vi "lab2_3.vi"() -> ()   [LabVIEW 2026]
uses:
  <vilib>/eio/EIONode/EIONode.xnode
  <vilib>/rvi/eio/common/nirviEmuTemplateMethod_errors.vi
panel:
  out "Mean X":fxp<+/-,64,33>
  out "AccelerationZ Now":i16
  out "AccelerationZ Max":i16
  out "AccelerationY Max":i16
  out "AccelerationY Now":i16
  out "AccelerationX Max":i16
  out "AccelerationX Now":i16
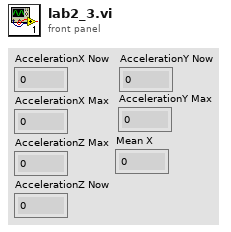
[diagram p1: front panel]
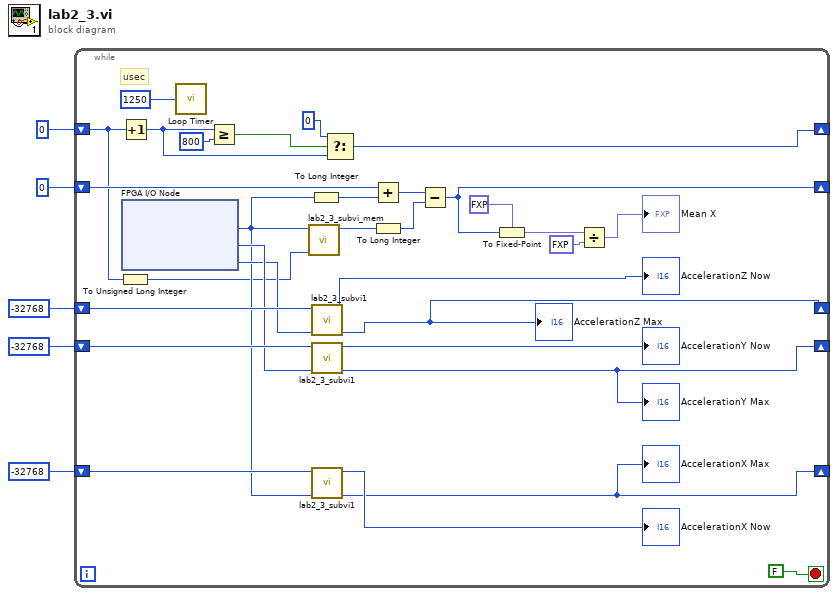
[diagram p0: block diagram]
diagram:
  n1 = while {
    shift-right: [w25] -> _
    shift-left: i16 -32768 ("x") -> [w30]
    shift-right: [w32] -> _
    shift-left: i16 -32768 ("x") -> [w34]
    shift-right: [w26] -> _
    shift-left: i16 -32768 ("x") -> [w31]
    shift-right: [w13] -> _
    shift-left: 0 ("x") -> [w23]
    shift-right: [w7] -> _
    shift-left: 0 ("x") -> [w6]
    stop <- FALSE stop-if-true
    # "usec"
    n2 = To Unsigned Long Integer(number=w6) -> (unsigned 32bit integer=w14:u32)
    n3 = Increment(x=w6) -> (x+1=w8:i32)
    n4 = xnode "FPGA I/O Node"() -> ("AccelerationX"=w21:i16, "AccelerationY"=w29:i16, "AccelerationZ"=w28:i16)  [unwired: 3 in, 3 out]
    n5 = call "Loop Timer"("Count(uSec)"=u32 1250) -> ()  [unwired: 1 out]
    n6 = Greater Or Equal?(x=w8, y=800) -> (x >= y?=w16:bool)
    n7 = call "lab2_3_subvi_mem.vi"("Address"=w14, "Data In"=w21) -> ("Last Value"=w19:i16)  [unwired: 9 in]
    n8 = To Long Integer(number=w21) -> (32bit integer=w22:i32)
    n9 = call "lab2_3_subvi1.vi"("Acc in"=w28, "Acc prev"=w30) -> ("Acceleration Max"=w25:i16, "Acceleration Now"=→"AccelerationZ Now":i16)  [unwired: 8 in]
    "AccelerationZ Max" <- w25
    n10 = call "lab2_3_subvi1.vi"("Acc in"=w29, "Acc prev"=w31) -> ("Acceleration Max"=w26:i16, "Acceleration Now"=→"AccelerationY Now":i16)  [unwired: 8 in]
    "AccelerationY Max" <- w26
    n11 = call "lab2_3_subvi1.vi"("Acc in"=w21, "Acc prev"=w34) -> ("Acceleration Max"=w32:i16, "Acceleration Now"=→"AccelerationX Now":i16)  [unwired: 8 in]
    "AccelerationX Max" <- w32
    n12 = Select(t=0, s=w16, f=w8) -> (s? t:f=w7:i32)
    n13 = Add(x=w23, y=w22) -> (x+y=w20:i32)
    n14 = To Long Integer(number=w19) -> (32bit integer=w18:i32)
    n15 = Subtract(x=w20, y=w18) -> (x-y=w13:i32)
    n16 = To Fixed-Point(fixed-point type=fxp<+/-,32,16> 30.0, number=w13) -> (fixed-point=w11:fxp<+/-,32,16>)
    n17 = Divide(x=w11, y=fxp<+/-,32,16> 800.0) -> (x/y=→"Mean X":fxp<+/-,64,33>)
  }
